vi "Update CAN Status.vi"(8 "error in (no error)":errorcluster, 11 "CAN_Writer_NIXNET_Plugin in":refnum<class "CAN_Writer_CANsub_Plugin.lvclass">) -> (0 "error out":errorcluster, 3 "CAN_Writer_NIXNET_Plugin out":refnum<class "CAN_Writer_CANsub_Plugin.lvclass">)   [LabVIEW 2021, in "CAN_Writer_CANsub_Plugin.lvclass"]
uses:
  CAN_Writer_CANsub_Plugin.lvclass
  CAN_Writer_CANsub_Plugin.lvclass/CAN_Writer_CANsub_Plugin.ctl
  <vilib>/CIF Foundation/CIF XNET CAN RW/XNET CAN RW.lvclass
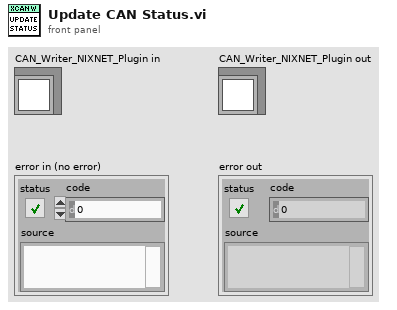
[diagram p1: front panel]
types:
  T1 = typedef "CAN_RW_CORE.lvclass/CAN Status.ctl" = cluster{"Comm State":T2, "Last Error":T3, "RX Error Counter":u8, "TX Error Counter":u8}
  T2 = typedef "CAN_RW_CORE.lvclass/Communication State.ctl" = enum16{"Error Active", "Error Passive", "Bus Off"}
  T3 = typedef "CAN_RW_CORE.lvclass/Last Error.ctl" = enum16{"None", "Stuff", "Form", "Ack", "Bit1", "Bit0", "CRC", "Unknown"}
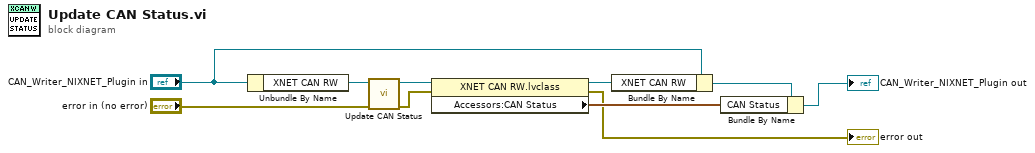
[diagram p0: block diagram]
diagram:
  n1 = Unbundle By Name("CAN_Writer_NIXNET_Plugin in") -> ("XNET CAN RW"=w8:refnum<class "XNET CAN RW.lvclass">)
  n2 = call <vilib>:"Update CAN Status.vi"("error in (no error)"="error in (no error)", "XNET CAN RW in"=w8) -> ("error out"=w6:errorcluster, "XNET CAN RW out"=w7:refnum<class "XNET CAN RW.lvclass">)  [unwired: 8 in]
  n3 = property class="XNET CAN RW.lvclass"(reference=w7, error in=w6) -> (reference out=w5:refnum<class "XNET CAN RW.lvclass">, error out=→"error out":errorcluster, "Accessors:CAN Status"=w3:T1)
  n4 = Bundle By Name(cluster="CAN_Writer_NIXNET_Plugin in", "XNET CAN RW"=w5) -> (w4:refnum<class "CAN_Writer_CANsub_Plugin.lvclass">)
  n5 = Bundle By Name(cluster=w4, "CAN Status"=w3) -> (→"CAN_Writer_NIXNET_Plugin out":refnum<class "CAN_Writer_CANsub_Plugin.lvclass">)
